vi "BoolCmd_Multiplexor.vi"(6 "Command Cancel":bool, 7 "Ready":bool=TRUE, 8 "Command 4":bool, 9 "Command 3":bool, 10 "Command 2":bool, 11 "Command 1":bool) -> (0 "Do Command 4":bool, 1 "Do Command 3":bool, 2 "Do Command 2":bool, 3 "Do Command 1":bool, 4 "Do Cancel":bool)   [LabVIEW 2019, in "Trajectory_Library.lvlib"]
uses:
  Trajectory_Library.lvlib
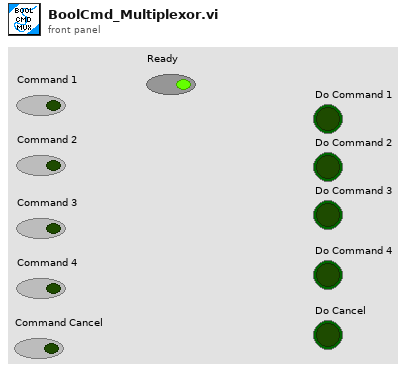
[diagram p1: front panel]
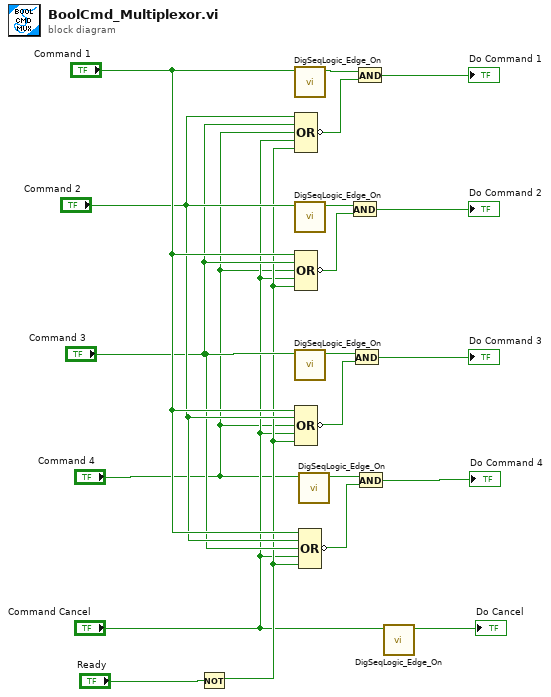
[diagram p0: block diagram]
diagram:
  n1 = Not(x="Ready") -> (.not. x?=w3:bool)
  n2 = call "DigSeqLogic_Edge_On.vi"("Input"="Command 1") -> ("On Edge"=w20:bool)  [unwired: 10 in]
  n3 = Compound Arithmetic op=OR("Command 2", "Command 3", "Command 4", "Command Cancel", w3) -> (invert w19:bool)
  n4 = call "DigSeqLogic_Edge_On.vi"("Input"="Command 2") -> ("On Edge"=w17:bool)  [unwired: 10 in]
  n5 = Compound Arithmetic op=OR("Command 1", "Command 3", "Command 4", "Command Cancel", w3) -> (invert w16:bool)
  n6 = call "DigSeqLogic_Edge_On.vi"("Input"="Command 3") -> ("On Edge"=w15:bool)  [unwired: 10 in]
  n7 = Compound Arithmetic op=OR("Command 1", "Command 2", "Command 4", "Command Cancel", w3) -> (invert w14:bool)
  n8 = call "DigSeqLogic_Edge_On.vi"("Input"="Command 4") -> ("On Edge"=w9:bool)  [unwired: 10 in]
  n9 = Compound Arithmetic op=OR("Command 1", "Command 2", "Command 3", "Command Cancel", w3) -> (invert w8:bool)
  n10 = And(x=w17, y=w16) -> (x .and. y?=→"Do Command 2":bool)
  n11 = And(x=w15, y=w14) -> (x .and. y?=→"Do Command 3":bool)
  n12 = And(x=w20, y=w19) -> (x .and. y?=→"Do Command 1":bool)
  n13 = And(x=w9, y=w8) -> (x .and. y?=→"Do Command 4":bool)
  n14 = call "DigSeqLogic_Edge_On.vi"("Input"="Command Cancel") -> ("On Edge"=→"Do Cancel":bool)  [unwired: 10 in]
